vi "Reset Stats CIF Subscriber.vi"(8 "error in (no error)":errorcluster, 11 "Subscriber Reference":T1 {"refnum" format="%.0x"}) -> (0 "error out":errorcluster)   [LabVIEW 2021, in "Iceoryx.lvlib"]
uses:
  Iceoryx.lvlib
  SubVIs/Convert Error Core.vi
  Refnum/Typedef/CIF Subscriber Refnum.ctl
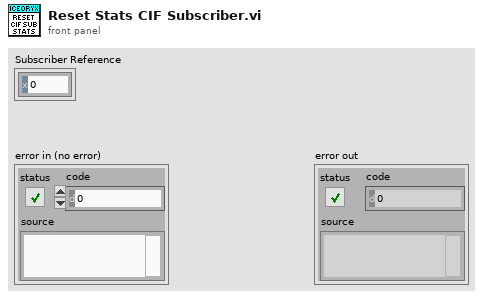
[diagram p1: front panel]
types:
  T1 = typedef "Iceoryx.lvlib/CIF Subscriber Refnum.ctl" = cluster{"refnum":u64, "CIF Sub":enum8{"cifsub"}}
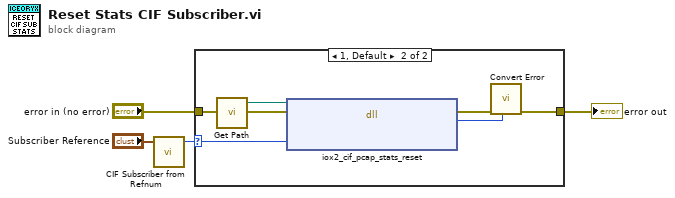
[diagram p0: block diagram]
diagram:
  n1 = call "CIF Subscriber from Refnum.vi"("CIF Subscriber Refnum"="Subscriber Reference") -> ("CIF Subscriber U64"=w1:u64)  [unwired: 4 in]
  n2 = case shown="1, Default" w1 {
    selector: w1 -> [_ w8]
    tunnel: "error in (no error)" -> [w5 w7]
    tunnel: [w5 w6] -> w2
    frame 0 {
    }
    frame 1, Default {
      n3 = call "Get Path.vi"() -> ("libiox2_cif path"=w11:path)  [unwired: 4 in]
      n4 = dll-call lib="D:/dev/iceoryx2_lvwrapper/dist/iox2_cif.dll" fn="iox2_cif_pcap_stats_reset"(path in=w11, error in=w7, "subscriber"=w8) -> (error out=w10:errorcluster, "return type"=w9:i32)  [unwired: 2 in, 1 out]
      n5 = call "Convert Error.vi"("return type"=w9, "error in (no error)"=w10) -> ("error out"=w6:errorcluster)  [unwired: 9 in]
    }
  }
  "error out" <- w2
